vi "CE SEM Mask.vi"(8 "error in (no error)":errorcluster, 11 "SA Measurement in":refnum<class "SA Measurement.lvclass">) -> (0 "error out":errorcluster, 3 "SA Measurement out":refnum<class "SA Measurement.lvclass">)   [LabVIEW 2023, in "Spectrum Analyzer.lvlib" / "SA Measurement.lvclass"]
uses:
  SA Measurement.lvclass
  SA Measurement.lvclass/SA Measurement.ctl
  Keysight 9020A/Keysight 9020A.lvclass
  TYPE DEFINITION/TYPE Limit Line Setting Table.ctl
  Spectrum Analyzer.lvlib
  Interface_Spectrum/Interface_Spectrum.lvclass
  D:/Project/IST013_CE Conduction Measurement/IST013-CE-Condcuted-Measurement/src/Spectrum Analyzer/Interface_Spectrum/Interface_Spectrum.lvclass
panel:
  out "Pass?":bool
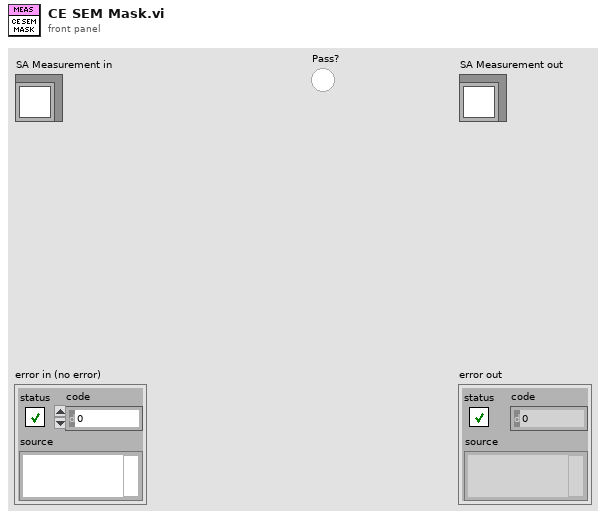
[diagram p1: front panel]
types:
  T1 = typedef "Spectrum Analyzer.lvlib/TYPE Limit Line Setting Table.ctl" = cluster{"Limit Line Index":i32, "Frequency Table":dbl[], "Amplitude Table":dbl[], "Name":string}
  T2 = typedef "Spectrum Analyzer.lvlib/TYPE Mask Table for SEM.ctl" = map{enum16{"-10dBm Upper", "-10dBm Lower"}, map{dbl, map{i32, cluster{"Freq":dbl, "Limit":dbl, "dBc Applied?":bool}[]}}}
  T3 = map{dbl, map{i32, cluster{"Freq":dbl, "Limit":dbl, "dBc Applied?":bool}[]}}
  T4 = map{i32, cluster{"Freq":dbl, "Limit":dbl, "dBc Applied?":bool}[]}
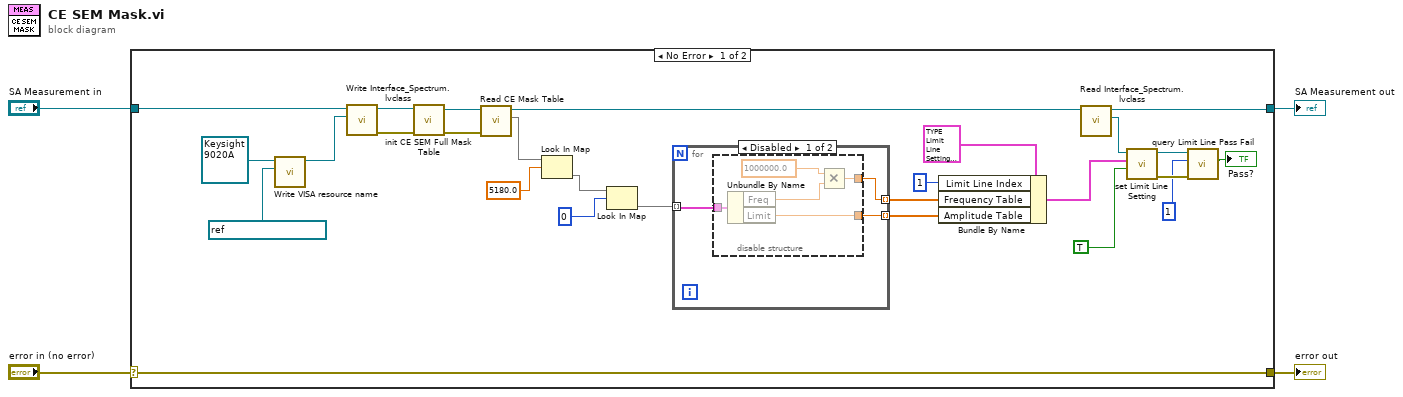
[diagram p0: block diagram]
diagram:
  n1 = case shown="No Error" "error in (no error)" {
    selector: "error in (no error)" -> [w31 w41]
    tunnel: [w31 w41] -> w3
    tunnel: [w12 w40] -> w1
    tunnel: "SA Measurement in" -> [w27 w40]
    frame No Error {
      n2 = call "Write VISA resource name.vi"("VISA resource name"=refnum<visa-resource-name> "GPIB0::18::INSTR", "Keysight 9020A in"=refnum<class "Keysight 9020A.lvclass"> refnum ("Spectrum Analyzer.lvlib:Keysight 9020A.lvclass")) -> ("Keysight 9020A out"=w28:refnum<class "Keysight 9020A.lvclass">)  [unwired: 8 in, 1 out]
      n3 = call "Write Interface_Spectrum.lvclass.vi"("Interface_Spectrum.lvclass"=w28, "SA Measurement in"=w27) -> ("error out"=w25:errorcluster, "SA Measurement out"=w26:refnum<class "SA Measurement.lvclass">)  [unwired: 8 in]
      n4 = call "init CE SEM Full Mask Table.vi"("error in (no error)"=w25, "SA Measurement in"=w26) -> ("error out"=w23:errorcluster, "SA Measurement out"=w24:refnum<class "SA Measurement.lvclass">)  [unwired: 8 in]
      n5 = call "Read CE Mask Table.vi"("error in (no error)"=w23, "SA Measurement in"=w24) -> ("Mask Table"=w22:T2, "SA Measurement out"=w13:refnum<class "SA Measurement.lvclass">)  [unwired: 7 in, 1 out]
      n6 = Look In Map(map=w22, key=5180.0) -> (value=w20:T3)  [unwired: 1 in, 1 out]
      n7 = Look In Map(map=w20, key=0) -> (value=w18:T4)  [unwired: 1 in, 1 out]
      n8 = for {
        tunnel: w18 -> [w34] mode=indexing
        tunnel: [w32] -> w15 mode=indexing
        tunnel: [w33] -> w14 mode=indexing
        n9 = disable-structure shown="Disabled" {
          disable-tunnel: w34 -> [w39 _]
          disable-tunnel: [w38 _] -> w33
          disable-tunnel: [w35 _] -> w32
          frame Disabled {
            n10 = Unbundle By Name(w39) -> ("Freq"=w37:dbl, "Limit"=w38:dbl)
            n11 = Multiply(x=1000000.0, y=w37) -> (x*y=w35:dbl)
          }
          frame Enabled {
          }
        }
      }
      n12 = Bundle By Name(cluster=T1 {"Limit Line Index"=1, "Frequency Table"=[1000000000.0, 2000000000.0, 3000000000.0], "Amplitude Table"=[-60.0, -50.0, -40.0], "Name"=""} ("Limit Line Setting"), "Limit Line Index"=1, "Frequency Table"=w15, "Amplitude Table"=w14) -> (w10:T1)
      n13 = call "Read Interface_Spectrum.lvclass.vi"("SA Measurement in"=w13) -> ("Interface_Spectrum.lvclass"=w11:refnum<class "Interface_Spectrum.lvclass">, "SA Measurement out"=w12:refnum<class "SA Measurement.lvclass">)  [unwired: 8 in, 1 out]
      n14 = call-dynamic "set Limit Line Setting.vi"("Turn On?"=TRUE, "Limit Line Setting"=w10, "Interface_Spectrum in"=w11) -> ("error out"=w7:errorcluster, "Interface_Spectrum out"=w8:refnum<class "Interface_Spectrum.lvclass">)  [unwired: 7 in]
      n15 = call-dynamic "query Limit Line Pass Fail.vi"("error in (no error)"=w7, "Limit Line Index"=1, "Interface_Spectrum in"=w8) -> ("Pass?"=→"Pass?":bool)  [unwired: 6 in, 2 out]
    }
    frame Error {
    }
  }
  "error out" <- w3
  "SA Measurement out" <- w1
